vi "PointNode_Create.vi"(0 "reference":refnum<class "PointNode.lvclass">, 5 "error in (no error)":errorcluster) -> (14 "reference out":refnum<class "PointNode.lvclass">, 19 "error out":errorcluster)   [LabVIEW 2020, in "PointNode.lvclass"]
doc: "Creates and initializes a new PointNode object.\n\nThis object should be destroyed using a PointNode destructor VI or a virtual base class destructor VI.\n\n[GOOP 2.1]"
uses:
  <resource>/Framework/Providers/Open_GDS/UML/PointNode_class/PointNode.lvclass
  C:/Program Files (x86)/National Instruments/LabVIEW 2020/resource/Framework/Providers/Open_GDS/UML/AbstractNode_class/AbstractNode.lvclass
  <resource>/Framework/Providers/Open_GDS/UML/General/Point/Point Point2D.ctl
  <resource>/Framework/Providers/Open_GDS/UML/AbstractNode_class/AbstractNode.lvclass
panel:
  # "The input reference should only\nbe wired when this method is called\nby a sub class constructor."
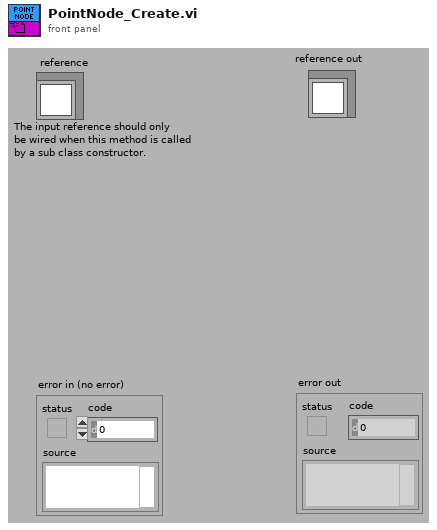
[diagram p1: front panel]
types:
  T1 = typedef "Point Point2D.ctl" = cluster{"x":dbl, "y":dbl}
  T2 = typedef "PointNode.lvclass/ObjectAttributes.ctl" = cluster{"point":T1}
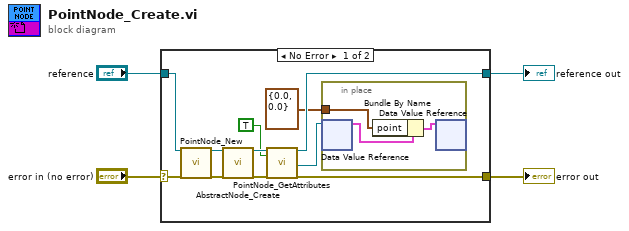
[diagram p0: block diagram]
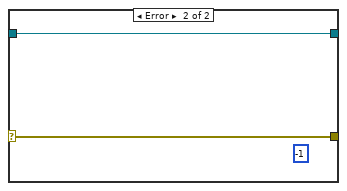
[diagram p2: hidden frame]
diagram:
  n1 = case shown="No Error" "error in (no error)" {
    selector: "error in (no error)" -> [w15 w20]
    tunnel: [w9 w19] -> w4
    tunnel: [w8 w20] -> w3
    tunnel: "reference" -> [w14 w19]
    frame No Error {
      n2 = call <resource>:"PointNode_New.vi"("reference in"=w14, "error in (no error)"=w15) -> ("reference out"=w11:refnum<class "PointNode.lvclass">, "error out"=w13:errorcluster)  [unwired: 2 in, 14 out]
      n3 = call <resource>:"AbstractNode_Create.vi"("reference"=w11, "error in (no error)"=w13) -> ("reference out"=w10:refnum<class "PointNode.lvclass">, "error out"=w12:errorcluster)  [unwired: 1 in, 15 out]
      n4 = call <resource>:"PointNode_GetAttributes.vi"("reference in"=w10, "OnlyGetDvrReference(False)"=TRUE, "error in (no error)"=w12) -> ("reference out"=w9:refnum<class "PointNode.lvclass">, "DataRef"=w6:refnum<data-value>, "error out"=w8:errorcluster)  [unwired: 13 in, 1 out]
      n5 = in-place {
        in-place-border: T1 {"x"=0.0, "y"=0.0} ("point") -> [w17]
        n6 = in-place-dvr #1(w6) -> (w18:T2)  [unwired: 1 out]
        n7 = Bundle By Name(cluster=w18, "point"=w17) -> (w16:T2)
        n8 = in-place-dvr #1(w16) -> ()  [unwired: 2 out]
      }
    }
    frame Error {
      (unwired) -1 ("Nr of open handles")
    }
  }
  "error out" <- w3
  "reference out" <- w4
